vi "VIH Project Tree - Relink File.vi"(6 "Ena Dialog Message (T)":bool=TRUE, 8 "error in":errorcluster, 9 "New File Path":path, 10 "Tree Item Tag":string, 11 "Project Tree":T1) -> (0 "error out":errorcluster, 1 "New File Path out":path, 2 "New Tree Item Tag":string, 3 "dup Project Tree":T1)   [LabVIEW 2014]
doc: "::: VI Helpeks :::\nCopyright (c) 2000-2026 Konstantin Shifershteyn. All rights reserved."
uses:
  VIH Project Tree Typedef - Tree Refnum.ctl
panel:
  # "VI Helpeks\nCopyright (c) 2012-2026 Konstantin Shifershteyn"
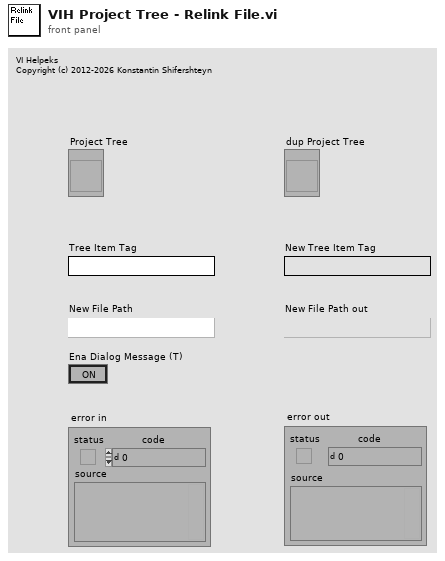
[diagram p1: front panel]
types:
  T1 = typedef "VIH Project Tree Typedef - Tree Refnum.ctl" = refnum<vi>
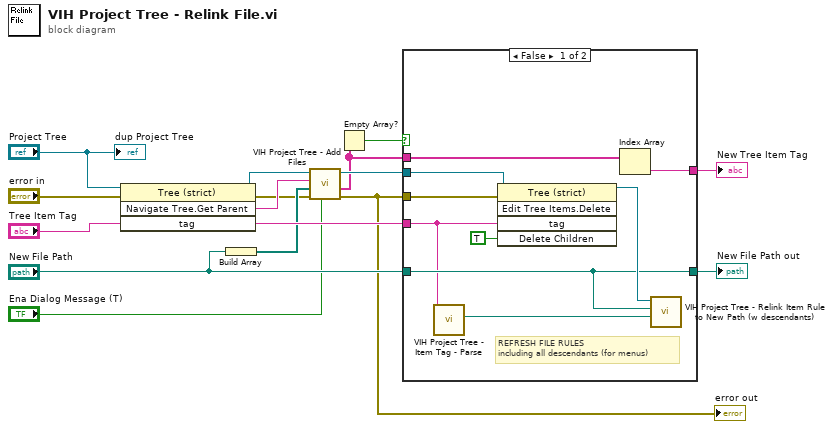
[diagram p0: block diagram]
diagram:
  n1 = invoke class="Tree (strict)" method="Navigate Tree.Get Parent"(reference="Project Tree", error in="error in", "tag"="Tree Item Tag") -> (reference out=w10:T1, error out=w7:errorcluster, "Navigate Tree:Get Parent"=w9:string)  [unwired: 1 in, 1 out]
  n2 = Build Array("New File Path") -> (w8:path[])
  n3 = call "VIH Project Tree - Add Files.vi"("Ena dialog message (F)"="Ena Dialog Message (T)", "error in"=w7, "File Paths"=w8, "Tree Parent Tag"=w9, "Project Tree"=w10) -> ("error out"=w1:errorcluster, "Top-level Item Tags"=w3:string[], "dup Project Tree"=w6:T1)  [unwired: 3 in, 1 out]
  "error out" <- w1
  n4 = Empty Array?(array=w3) -> (empty?=w4:bool)
  n5 = case shown="False" w4 {
    tunnel: "Tree Item Tag" -> [w16 _]
    tunnel: w1 -> [w23 _]
    tunnel: w6 -> [w22 _]
    tunnel: w3 -> [w21 _]
    tunnel: "New File Path" -> [w18 _]
    tunnel: [w20 _] -> w14
    tunnel: [w18 _] -> w13
    frame False {
      # "REFRESH FILE RULES\nincluding all descendants (for menus)"
      n6 = call "VIH Project Tree - Item Tag - Parse.vi"("Tree Item Tag"=w16) -> ("Item File Path"=w17:path)  [unwired: 8 in, 2 out]
      n7 = invoke class="Tree (strict)" method="Edit Tree Items.Delete"(reference=w22, error in=w23, "tag"=w16, "Delete Children"=TRUE) -> (reference out=w19:T1)  [unwired: 1 in, 4 out]
      n8 = Index Array(array=w21) -> (element=w20:string)  [unwired: 1 in]
      n9 = call "VIH Project Tree - Relink Item Rule to New Path (w descendants).vi"("Old Item Path"=w17, "New Item Path"=w18, "Project Tree"=w19) -> ()  [unwired: 5 in, 4 out]
    }
    frame True {
    }
  }
  "New Tree Item Tag" <- w14
  "New File Path out" <- w13
  "dup Project Tree" <- "Project Tree"
